vi "Do Request.vi"(7 "Processing In":refnum<class "Processing.lvclass">, 11 "DebugHTTPController in":refnum<class "DebugHTTPController.lvclass">) -> (0 "error out":errorcluster, 5 "Processing":refnum<class "Processing.lvclass">)   [LabVIEW 2020, in "Volatus.lvlib" / "DebugHTTPController.lvclass"]
doc: "A controller's main job is to respond to a request by generating a response. The response value must be specified by calling Set Response.vi on the Processing class that's passed through the VI otherwise an error will be generated.\n\nThere are several helpers available for common response types:\nGenerating HTML content programmatically - Create Basic Response.vi\nStreaming a file from disk - Create File Response.vi\nRedirecting the user to another URL - Create Redirect Response.vi\n\nFile responses are streamed in chunks and do not load the entire file into memory at once to send in the response which allows serving large files more efficiently."
uses:
  DebugHTTPController.lvclass
  lv-http-server/HTTP Server/Processing/Processing.lvclass
  DebugHTTPController.lvclass/DebugHTTPController.ctl
  lv-http-server/HTTP Server/Processing/Processing.lvclass/Processing.ctl
  PathValue/PathValue.lvclass
  C:/dev/lv20CE/relink/lv-promises/Promises/Value/Value.lvclass
  PathValue/PathValue.lvclass/PathValue.ctl
  MessageQ/MessageQ.lvclass/MessageQ.ctl
  StatusTreeValue/StatusTreeValue.lvclass
  lv-http-util/HTTP Utils/File Response/File Response.lvclass
  C:/dev/lv20CE/relink/lv-http-util/HTTP Utils/Response/Response.lvclass
  lv-http-util/HTTP Utils/Request/Get Target URI.vi
  lv-stream/stream/URI/Get Path.vi
  MessageQ/MessageQ.lvclass
  lv-http-util/HTTP Utils/Response/Response.lvclass
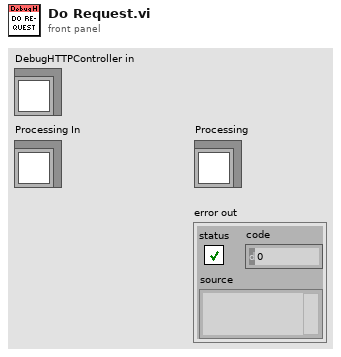
[diagram p1: front panel]
types:
  T1 = typedef "Volatus.lvlib/Module Status.ctl" = cluster{"Hierarchy":string[], "State":T2, "Substatus":map{string, string}, "Metrics":map{string, dbl}}
  T2 = typedef "Volatus.lvlib/Module.lvclass/State.ctl" = enum16{"Unknown", "Launched", "Starting", "Running", "Stopping", "Stopped", "Error - Starting", "Error - Run", "Error - Stopping"}
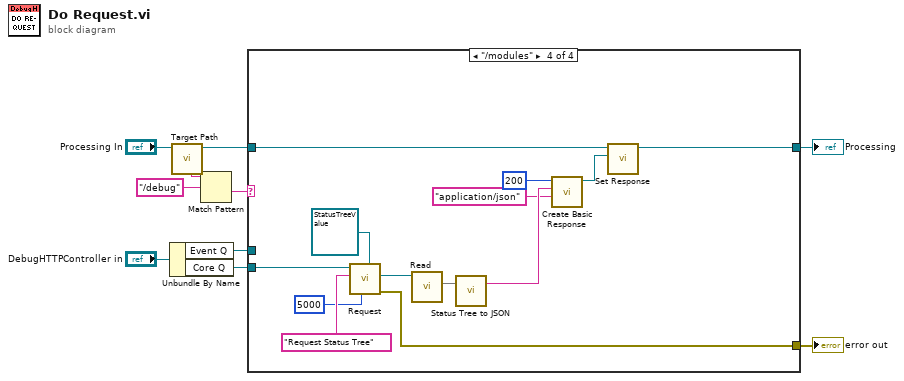
[diagram p0: block diagram]
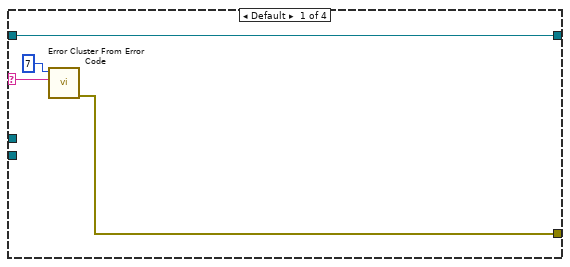
[diagram p2: hidden frame]
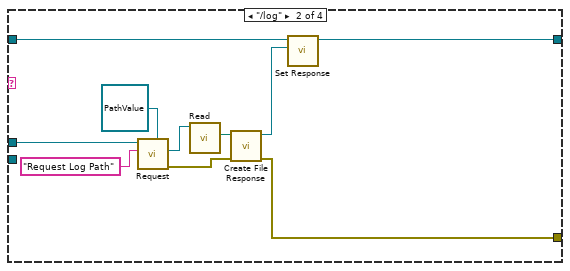
[diagram p3: hidden frame]
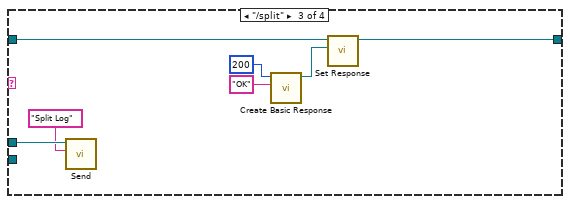
[diagram p4: hidden frame]
diagram:
  n1 = Unbundle By Name("DebugHTTPController in") -> ("Event Q"=w2:refnum<class "MessageQ.lvclass">, "Core Q"=w1:refnum<class "MessageQ.lvclass">)
  n2 = call "Target Path.vi"("Processing in"="Processing In") -> ("Processing out"=w6:refnum<class "Processing.lvclass">, "Target Path"=w10:string)  [unwired: 9 in]
  n3 = Match Pattern(string=w10, regular expression="/debug") -> (after substring=w7:string)  [unwired: 1 in, 3 out]
  n4 = case shown="\"/modules\"" w7 {
    selector: w7 -> [w14 _ _ _]
    tunnel: w6 -> [w12 w24 w31 w35]
    tunnel: [w12 w16 w26 w33] -> w5
    tunnel: [w11 w17 _ w40] -> w4
    tunnel: w2 -> [_ w23 w30 _]
    tunnel: w1 -> [_ _ _ w44]
    frame Default {
      n5 = call <vilib>:"Error Cluster From Error Code.vi"("error message (\"\")"=w14, "error code (0)"=7) -> ("error out"=w11:errorcluster)  [unwired: 7 in]
    }
    frame "/log" {
      n6 = call "Request.vi"("Response Value Type"=refnum<class "PathValue.lvclass"> refnum ("Volatus:PathValue.lvclass"), "ID"="Request Log Path", "MessageQ in"=w23) -> ("error out"=w18:errorcluster, "Response"=w20:refnum<class "PathValue.lvclass">)  [unwired: 6 in, 1 out]
      n7 = call "Read.vi"("PathValue in"=w20) -> ("Path"=w19:path)  [unwired: 10 in]
      n8 = call "Create File Response.vi"("error in (no error)"=w18, "Path"=w19) -> ("error out"=w17:errorcluster, "File Response out"=w15:refnum<class "File Response.lvclass">)  [unwired: 8 in]
      n9 = call "Set Response.vi"("Response"=w15, "Processing in"=w24) -> ("Processing out"=w16:refnum<class "Processing.lvclass">)  [unwired: 9 in]
    }
    frame "/split" {
      n10 = call "Send.vi"("ID"="Split Log", "MessageQ in"=w30) -> ()  [unwired: 8 in, 2 out]
      n11 = call "Create Basic Response.vi"("Payload"="OK", "Status Code"=u16 200) -> ("Response out"=w25:refnum<class "Response.lvclass">)  [unwired: 8 in, 1 out]
      n12 = call "Set Response.vi"("Response"=w25, "Processing in"=w31) -> ("Processing out"=w26:refnum<class "Processing.lvclass">)  [unwired: 9 in]
    }
    frame "/modules" {
      n13 = call "Request.vi"("Response Value Type"=refnum<class "StatusTreeValue.lvclass"> refnum ("Volatus:StatusTreeValue.lvclass"), "Timeout ms (1000)"=5000, "ID"="Request Status Tree", "MessageQ in"=w44) -> ("error out"=w40:errorcluster, "Response"=w41:refnum<class "StatusTreeValue.lvclass">)  [unwired: 5 in, 1 out]
      n14 = call "Read.vi"("StatusTreeValue in"=w41) -> ("Status Tree"=w39:map{string[], T1})  [unwired: 10 in]
      n15 = call "Status Tree to JSON.vi"("Status Tree"=w39) -> ("JSON"=w37:string)  [unwired: 6 in]
      n16 = call "Create Basic Response.vi"("Content-Type (text/plain)"="application/json", "Payload"=w37, "Status Code"=u16 200) -> ("Response out"=w34:refnum<class "Response.lvclass">)  [unwired: 7 in, 1 out]
      n17 = call "Set Response.vi"("Response"=w34, "Processing in"=w35) -> ("Processing out"=w33:refnum<class "Processing.lvclass">)  [unwired: 9 in]
    }
  }
  "error out" <- w4
  "Processing" <- w5
